vi "Write Channels.vi"(8 "error in (no error)":errorcluster, 10 "Channels":refnum<class "Abs_Type.lvclass">[](array[class]), 11 "CTI_Bus in":refnum<class "CTI_Bus.lvclass">) -> (0 "error out":errorcluster, 3 "CTI_Bus out":refnum<class "CTI_Bus.lvclass">)   [LabVIEW 2021, in "CTI_Bus.lvclass"]
uses:
  CTI_Bus.lvclass
  <vilib>/TSA/Abstract Data Classes/Abs_Types/Type/Abs_Type.lvclass
  CTI_Bus.lvclass/CTI_Bus.ctl
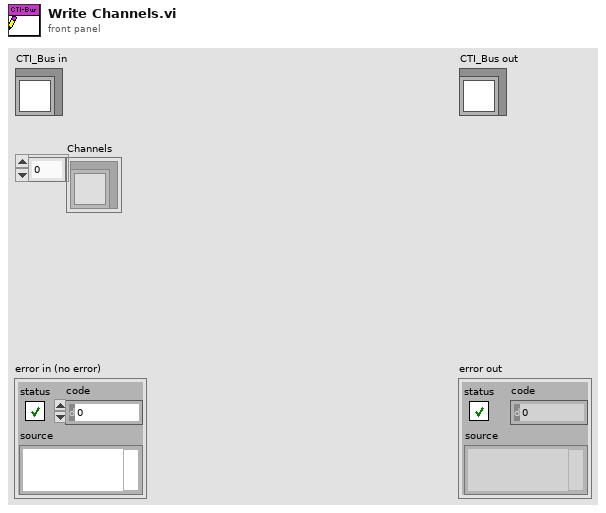
[diagram p1: front panel]
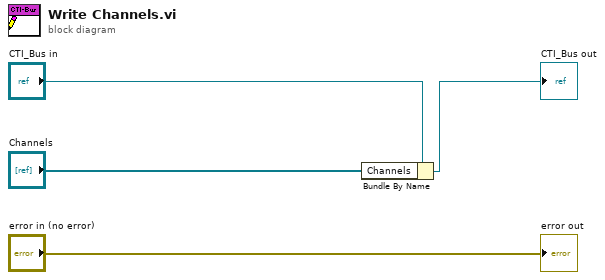
[diagram p0: block diagram]
diagram:
  n1 = Bundle By Name(cluster="CTI_Bus in", "Channels"="Channels") -> (→"CTI_Bus out":refnum<class "CTI_Bus.lvclass">)
  "error out" <- "error in (no error)"
